vi "DMM Read Ripple.vi"(0 "instrument handle":refnum<k15>, 11 "error in":errorcluster) -> (4 "instrument handle out":refnum<k15>, 6 "Ripple pp (V)":dbl, 8 "Ripple RMS (V)":dbl, 15 "error out":errorcluster)   [LabVIEW 2026]
doc: "Configures the NI-DMM session for a waveform voltage acquisition on the 10 V range at 100 kS/s and reads 20000 points (0.2 s). Ripple pp is max - min of the samples and Ripple RMS is their sample standard deviation (the AC part). Leaves the DMM in waveform mode and does not open or close the session."
uses:
  <vilib>/Analysis/NI_AALBase.lvlib
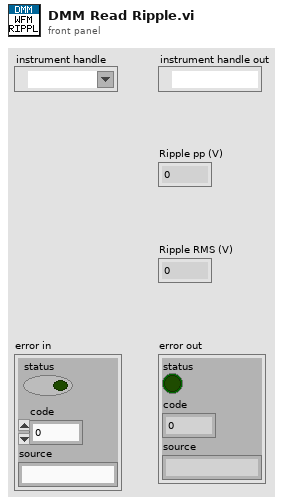
[diagram p1: front panel]
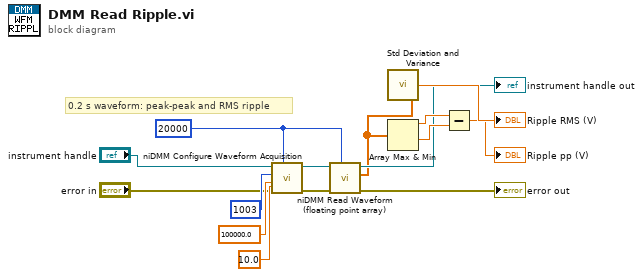
[diagram p0: block diagram]
diagram:
  w6 = 20000 ("Waveform Points")
  # "0.2 s waveform: peak-peak and RMS ripple"
  n1 = call <instrlib>:"niDMM Configure Waveform Acquisition.vi"("Range"=10.0, "Waveform Points"=w6, "error in (no error)"="error in", "Rate"=100000.0, "Function"=1003, "instrument handle"="instrument handle") -> ("error out"=w7:errorcluster, "instrument handle out"=w8:refnum<k15>)  [unwired: 4 in]
  n2 = call <instrlib>:"niDMM Read Waveform (floating point array).vi"("Number To Read"=w6, "error in (no error)"=w7, "instrument handle"=w8) -> ("error out"=→"error out":errorcluster, "Measurements Array"=w10:dbl[], "instrument handle out"=→"instrument handle out":refnum<k15>)  [unwired: 5 in, 1 out]
  n3 = call <vilib>:"Std Deviation and Variance.vi"("X"=w10) -> ("standard deviation"=→"Ripple RMS (V)":dbl)  [unwired: 1 in, 2 out]
  n4 = Array Max & Min(array=w10) -> (max value=w12:dbl, min value=w13:dbl)  [unwired: 2 out]
  n5 = Subtract(x=w12, y=w13) -> (x-y=→"Ripple pp (V)":dbl)
